vi "Iceoryx Channel Errors.vi"(8 "error in (no error)":errorcluster, 9 "String to Append":string, 10 "Error":T1, 11 "Insert Error":bool=TRUE) -> (0 "error out":errorcluster)   [LabVIEW 2021, in "CIF_Iceoryx_Chn.lvclass"]
uses:
  CIF_Iceoryx_Chn.lvclass
  Typedef/Iceoryx Channel Error.ctl
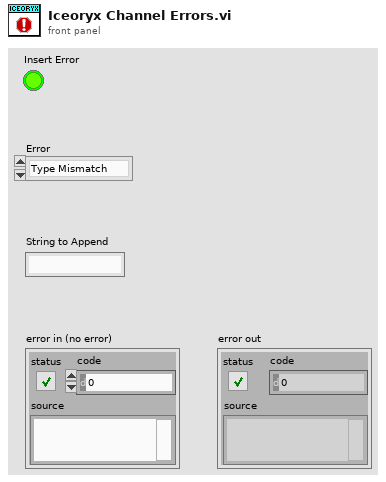
[diagram p1: front panel]
types:
  T1 = typedef "CIF_Iceoryx_Chn.lvclass/Iceoryx Channel Error.ctl" = enum16{"Type Mismatch", "Name Mismatch", "Override Required"}
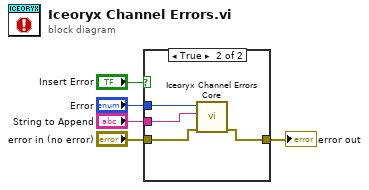
[diagram p0: block diagram]
diagram:
  n1 = case shown="True" "Insert Error" {
    tunnel: [w6 w7] -> w4
    tunnel: "error in (no error)" -> [w6 w8]
    tunnel: "Error" -> [_ w10]
    tunnel: "String to Append" -> [_ w9]
    frame False {
    }
    frame True {
      n2 = call "Iceoryx Channel Errors Core.vi"("error in (no error)"=w8, "String to Append"=w9, "Error"=w10) -> ("error out"=w7:errorcluster)  [unwired: 8 in]
    }
  }
  "error out" <- w4
